vi "Line Follower.vi"   [LabVIEW 2015, in "Roboter.lvrbt"]
uses:
  Roboter.lvrbt
  <vilib>/NXT/Block Support/NXT_OutputPort.ctl
  <vilib>/NXT/Block Support/NXT_InputPort.ctl
  <vilib>/NXT/Dual Mode Library/Sensors/Light_On.vi
  <vilib>/NXT/Dual Mode Library/Sensors/readNXTButton.vi
  <vilib>/NXT/NXTIO Xnodes/NXTIONodeSubVIs/NXTMoveMotors.vi
  <vilib>/NXT/NXTIO Xnodes/AddressXNode/NXTIOAddress.xnode
  <vilib>/NXT/Subs/LVHSConnector.ctl
  <vilib>/NXT/NXTIO Xnodes/NXTIOXNode/NXTIO.xnode
  <vilib>/NXT/LegoClasses/BrickReference/BrickReference.lvclass
types:
  T1 = typedef "NXT_OutputPort.ctl" = u8
  T2 = typedef "NXT_InputPort.ctl" = u32
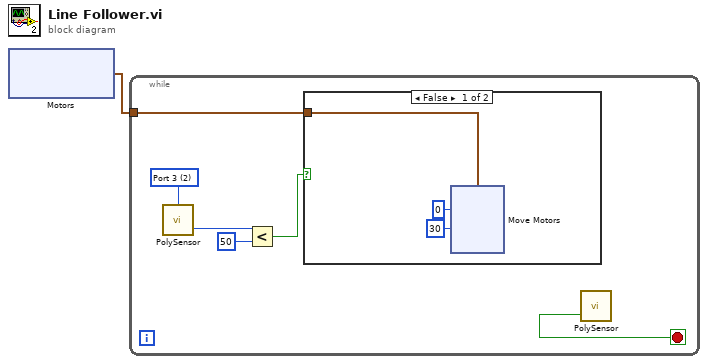
[diagram p0: block diagram]
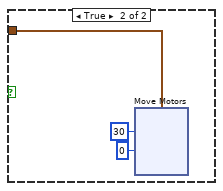
[diagram p2: hidden frame]
diagram:
  n1 = xnode "Motors"() -> ("Motor"=w1:cluster{"Port":T1, "Port":T1})
  n2 = while {
    tunnel: w1 -> [w5]
    stop <- w7 stop-if-true
    w6 = T2 2 items=["Port 1", "Port 2", "Port 3", "Port 4"] ("Port (Port 3)")
    n3 = call-poly <vilib>:"PolySensor.vi"("Port (Port 3)"=w6) -> ("Scaled Value"=w4:i16)  [unwired: 2 in, 1 out]
    n4 = Less?(x=w4, y=i16 50) -> (x < y?=w2:bool)
    n5 = case shown="False" w2 {
      tunnel: w5 -> [w10 w21]
      frame False {
        n6 = xnode "Move Motors"("Power/Speed 2"=i8 30, "Power/Speed 1"=i8 0, "Motors"=w10) -> ()  [unwired: 1 in, 1 out]
      }
      frame True {
        n7 = xnode "Move Motors"("Power/Speed 2"=i8 0, "Power/Speed 1"=i8 30, "Motors"=w21) -> ()  [unwired: 1 in, 1 out]
      }
    }
    n8 = call-poly <vilib>:"PolySensor.vi"() -> ("Yes/No"=w7:bool)  [unwired: 3 in, 1 out]
  }
